vi "INIT-Connect.vi"(8 "error in (no error)":errorcluster caption="错误输入（无错误）", 10 "database-path":path, 11 "Database_access 输入":refnum<class "Database_access.lvclass">) -> (0 "error out":errorcluster caption="错误输出", 3 "Database_access 输出":refnum<class "Database_access.lvclass">)   [LabVIEW 2025, in "Database_access.lvclass"]
uses:
  Database_access.lvclass
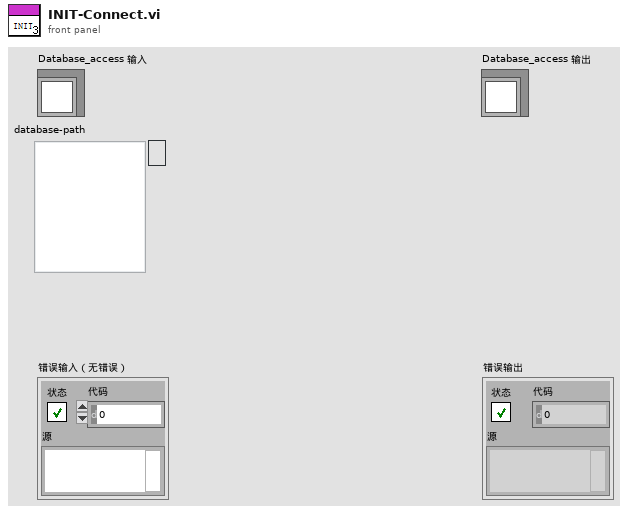
[diagram p1: front panel]
types:
  T1 = typedef "NI_Database_API.lvlib/Conn ObjectReference.ctl" = refnum<k1>
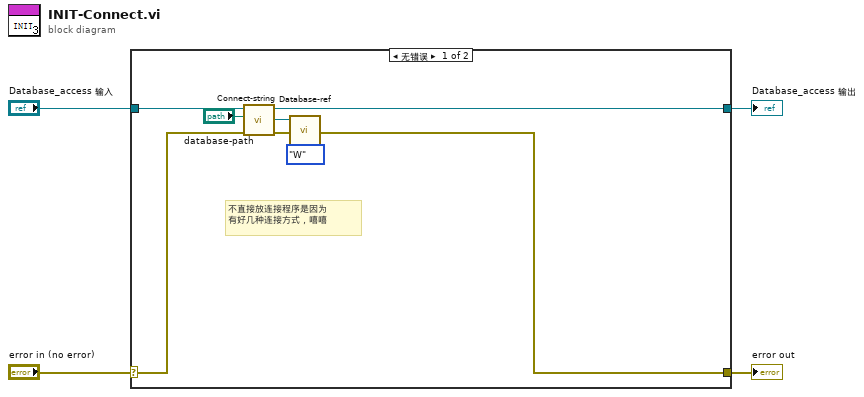
[diagram p0: block diagram]
diagram:
  n1 = case shown="无错误" "error in (no error)" {
    selector: "error in (no error)" -> [w8 w13]
    tunnel: [w7 w13] -> w3
    tunnel: [w10 w12] -> w1
    tunnel: "Database_access 输入" -> [w11 w12]
    frame No Error {
      # "不直接放连接程序是因为\n有好几种连接方式，嘻嘻"
      n2 = call-dynamic "Connect-string.vi"("error in (no error)"=w8, "database-path"="database-path", "Database_access 输入"=w11) -> ("error out"=w7:errorcluster, "connection reference"=w6:T1, "Database_access 输出"=w10:refnum<class "Database_access.lvclass">)  [unwired: 6 in]
      n3 = call "Database-ref.vi"("枚举"=enum16{"W", "R"}."W", "connection reference"=w6) -> ()  [unwired: 9 in, 1 out]
    }
    frame Error {
    }
  }
  "error out" <- w3
  "Database_access 输出" <- w1
